vi "RemoteVI Open Server.vi"(11 "error in":errorcluster) -> (15 "error out":errorcluster)   [LabVIEW 2020, in "RemoteVI.lvlib"]
doc: "Opens RemoteVI Server (..\\App\\RemoteVI Server.vi, the window that shares any window in a browser without code) and returns at once: if it is already open it is brought to the front, else it is opened and run. The Tools menu entry Tools > RemoteVI > Share in Browser calls it. Closing RemoteVI Server's window in LabVIEW keeps its shares running; open it again to see or stop them."
uses:
  RemoteVI.lvlib
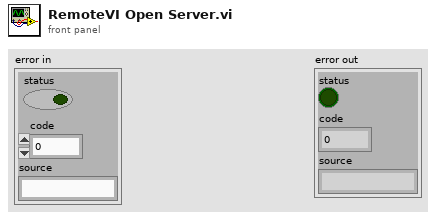
[diagram p1: front panel]
types:
  T1 = enum32{"Bad", "Idle", "Run top level", "Running"}
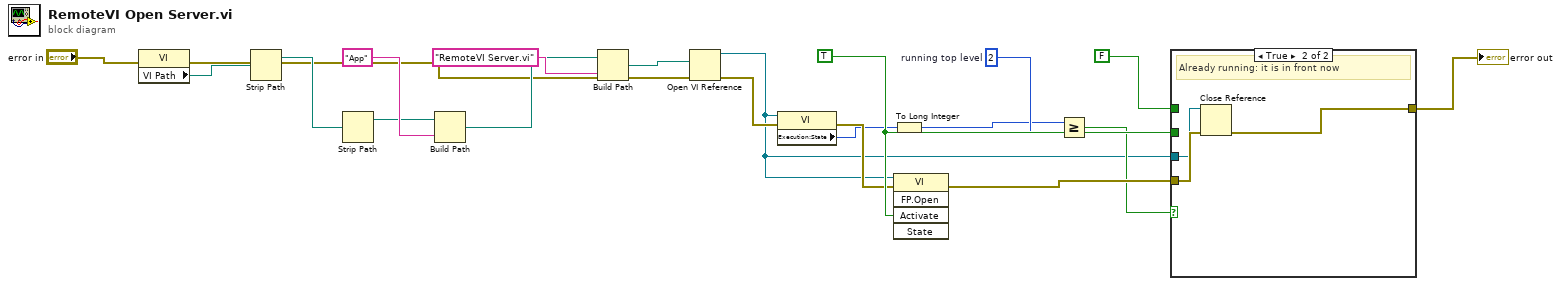
[diagram p0: block diagram]
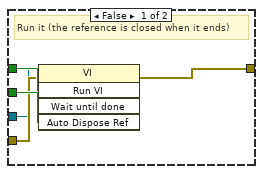
[diagram p2: hidden frame]
diagram:
  w17 = TRUE
  w15 = 2  # running top level
  n1 = property class="VI"(error in="error in") -> (error out=w2:errorcluster, "VI Path"=w3:path)  [unwired: 1 in, 1 out]
  n2 = Strip Path(path=w3) -> (stripped path=w4:path)  [unwired: 1 out]
  n3 = Strip Path(path=w4) -> (stripped path=w5:path)  [unwired: 1 out]
  n4 = Build Path(base path=w5, name or relative path="App") -> (appended path=w7:path)
  n5 = Build Path(base path=w7, name or relative path="RemoteVI Server.vi") -> (appended path=w9:path)
  n6 = Open VI Reference(vi path=w9, error in (no error)=w2) -> (vi reference=w10:refnum<vi>, error out=w11:errorcluster)  [unwired: 4 in]
  n7 = property class="VI"(reference=w10, error in=w11) -> (error out=w13:errorcluster, "Execution:State"=w12:T1)  [unwired: 1 out]
  n8 = To Long Integer(number=w12) -> (32bit integer=w14:i32)
  n9 = invoke class="VI" method="FP.Open"(reference=w10, error in=w13, "Activate"=w17) -> (error out=w19:errorcluster)  [unwired: 2 in, 4 out]
  n10 = Greater Or Equal?(x=w14, y=w15) -> (x >= y?=w16:bool)
  n11 = case shown="True" w16 {
    tunnel: FALSE -> [w23 _]
    tunnel: w17 -> [w24 _]
    tunnel: w10 -> [w21 w26]
    tunnel: w19 -> [w22 w27]
    tunnel: [w25 w28] -> w20
    frame False {
      # "Run it (the reference is closed when it ends)"
      n12 = invoke class="VI" method="Run VI"(reference=w21, error in=w22, "Wait until done"=w23, "Auto Dispose Ref"=w24) -> (error out=w25:errorcluster)  [unwired: 1 in, 4 out]
    }
    frame True {
      # "Already running: it is in front now"
      n13 = Close Reference(reference=w26, error in (no error)=w27) -> (error out=w28:errorcluster)
    }
  }
  "error out" <- w20
